vi "LinearQuadraticRegulator_New_ELMS.vi"(5 "States":i32, 6 "dt_Seconds":dbl=0.02, 7 "Inputs":i32, 8 "Relms":T2, 9 "Qelms":T2, 10 "B":T2, 11 "A":T2) -> (0 "Error":bool, 3 "LinearQuadraticRegulator":T1)   [LabVIEW 2019, in "Trajectory_Library.lvlib"]
doc: "Contains the controller coefficients and logic for a linear-quadratic regulator (LQR). LQRs use the control law u = K(r - x).\n \nFor more on the underlying math, read https://file.tavsys.net/control/controls-engineering-in-frc.pdf.\n\nConstructs a controller with the given coefficients and plant.\n\nInputs:\n - A -- Continuous system matrix of the plant being controlled.\n - B -- Continuous input matrix of the plant being controlled.\n - qelms -- The maximum desired error tolerance for each state.\n - relms -- The maximum desired control effort for each input.\n - dtSeconds -- Discretization timestep.\n\nOutputs:\n - LinearQuadraticRegulator -- controller data cluster\n - Error -- If TRUE, an error occured."
uses:
  Trajectory_Library.lvlib
  <vilib>/Analysis/Matrix/Datatypes/RealMatrix.ctl
  <vilib>/Analysis/Matrix/NI_Matrix.lvlib
  TypeDef/LINEAR_QUADRATIC_REGULATOR.ctl
panel:
  # "<States,States>"
  # "<States,Inputs>"
  # "<States,1>"
  # "<Inputs,1>"
  # "Ref State <States,1>"
  # "Comp and capped \noutput <Inputs,1>"
  # "Controller gain\n<Inputs,States>"
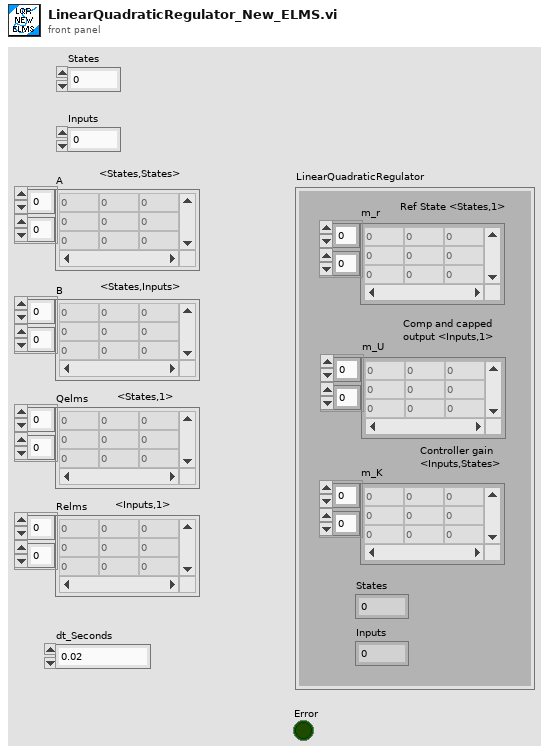
[diagram p1: front panel]
types:
  T1 = typedef "Trajectory_Library.lvlib/LINEAR_QUADRATIC_REGULATOR.ctl" = cluster{"m_r":T2, "m_U":T2, "m_K":T2, "States":i32, "Inputs":i32}
  T2 = typedef "NI_Matrix.lvlib/RealMatrix.ctl" = dbl[][]
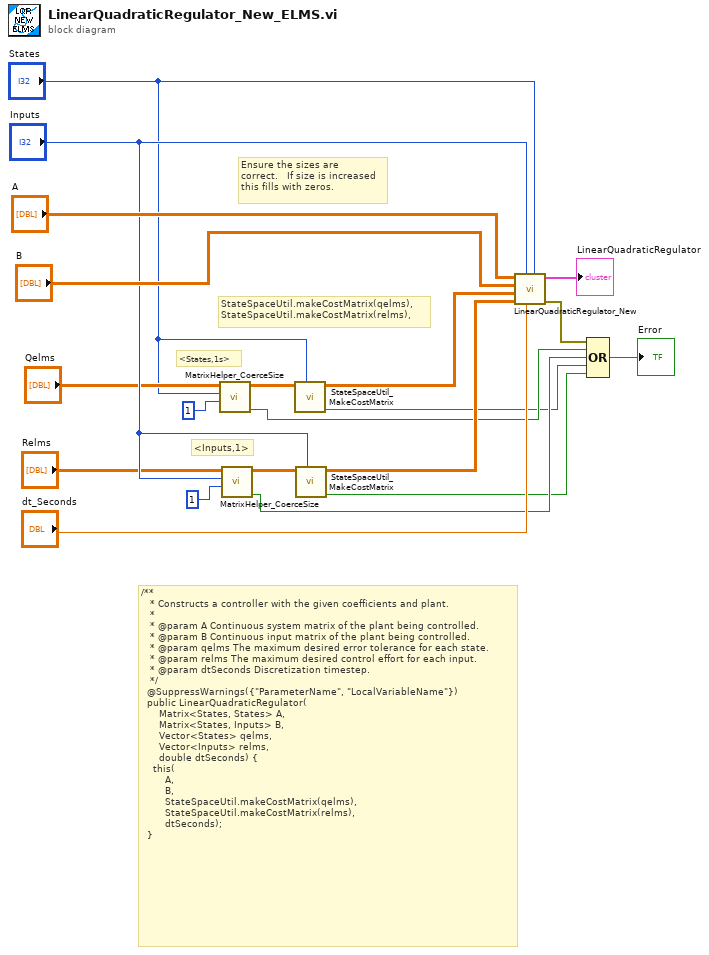
[diagram p0: block diagram]
diagram:
  # "StateSpaceUtil.makeCostMatrix(qelms),\nStateSpaceUtil.makeCostMatrix(relms),"
  # "<Inputs,1>"
  # "<States,1s>"
  # "Ensure the sizes are\ncorrect.   If size is increased \nthis fills with zeros."
  # "/**\n   * Constructs a controller with the given coefficients and plant.\n   *\n   * @param A Continuous system matrix of the plant being controlled.\n   * @param B Continuous input matrix of the plant being controlled.\n   * @param qelms The maximum desired error tolerance for each state.\n   * @param relms The maximum desired control effort for each input.\n   * @param dtSeconds Discretization timestep.\n   */\n  @SuppressWarnings({\"ParameterName\", \"LocalVariableName\"})\n  public LinearQuadraticRegulator(\n      Matrix<States, States> A,\n      Matrix<States, Inputs> B,\n      Vector<States> qelms,\n      Vector<Inputs> relms,\n      double dtSeconds) {\n    this(\n        A,\n        B,\n        StateSpaceUtil.makeCostMatrix(qelms),\n        StateSpaceUtil.makeCostMatrix(relms),\n        dtSeconds);\n  }"
  n1 = call "MatrixHelper_CoerceSize.vi"("Columns"=1 ("number of columns"), "Rows"="States", "input matrix"="Qelms") -> ("Coerced"=w4:bool, "output matrix"=w10:T2)  [unwired: 7 in]
  n2 = call "MatrixHelper_CoerceSize.vi"("Columns"=1 ("number of columns"), "Rows"="Inputs", "input matrix"="Relms") -> ("Coerced"=w3:bool, "output matrix"=w11:T2)  [unwired: 7 in]
  n3 = call "StateSpaceUtil_MakeCostMatrix.vi"("Elements"="States", "Costs"=w10) -> ("Sze Coerced"=w2:bool, "Costs Matrix"=w17:T2)  [unwired: 8 in]
  n4 = call "StateSpaceUtil_MakeCostMatrix.vi"("Elements"="Inputs", "Costs"=w11) -> ("Sze Coerced"=w1:bool, "Costs Matrix"=w16:T2)  [unwired: 8 in]
  n5 = call "LinearQuadraticRegulator_New.vi"("States"="States", "dt_Seconds"="dt_Seconds", "Inputs"="Inputs", "R"=w16, "Q"=w17, "B"="B", "A"="A") -> ("Error"=w5:errorcluster, "LinearQuadraticRegulator"=→"LinearQuadraticRegulator":T1)  [unwired: 3 in]
  n6 = Compound Arithmetic op=OR(w5, w4, w3, w2, w1) -> (→"Error":bool)
